vi "Condition_Eval_Logic.vi"(8 "error in (no error)":errorcluster={"status"=FALSE, "code"=0, "source"="\"\""}, 11 "Child ConditionResults":string) -> (0 "error out":errorcluster={"status"=FALSE, "code"=0, "source"="\"\""}, 2 "status ok":bool, 3 "ConditionResult":string)   [LabVIEW 2026]
doc: "INTENT: Combine AND/OR/NOT expressions. LOGIC: Apply three-valued logic preserving definitive false for AND and true for OR where valid; otherwise unknown."
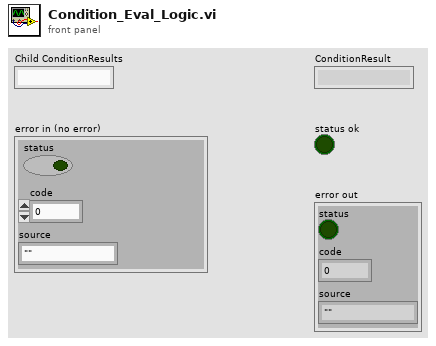
[diagram p1: front panel]
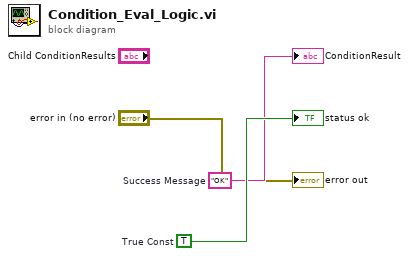
[diagram p0: block diagram]
diagram:
  w3 = TRUE  # True Const
  w2 = "OK"  # Success Message
  "ConditionResult" <- w2
  "status ok" <- w3
  "error out" <- "error in (no error)"
